vi "Test Client Alone With No Server.vi"(8 "error in (no error)":errorcluster) -> (0 "error out":errorcluster)   [LabVIEW 2019, in "RemoteControl.ZMQ.Tests.lvclass"]
uses:
  RemoteControl.ZMQ.Tests.lvclass
  C:/Program Files/National Instruments/LabVIEW 2019/user.lib/LevyLab/RemoteControl/RemoteControl/RemoteControl.lvclass
  <userlib>/LevyLab/RemoteControl/RemoteControl/RemoteControl.lvclass/RemoteControl.ctl
  <vilib>/numeric/Random Number (Range) U64.vi
  <vilib>/numeric/sub_Random U32.vi
  <vilib>/addons/_JKI Toolkits/Caraya/classes/Assert/Assert True.vi
  <userlib>/LevyLab/RemoteControl/RemoteControl/RemoteControl.lvclass
  <vilib>/addons/_JKI Toolkits/Caraya/classes/Assert/Assert.lvclass
  <vilib>/addons/_JKI Toolkits/Caraya/classes/Test/Test.lvclass
panel:
  out "code":i32
  out "Codes":i32[](array[numeric])
  in  "stop":bool
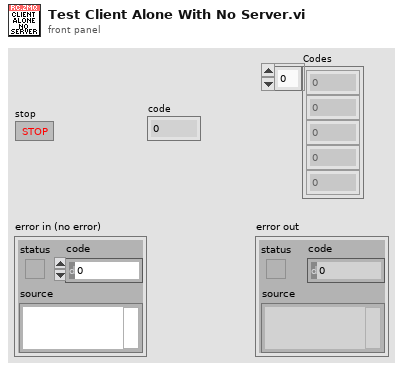
[diagram p1: front panel]
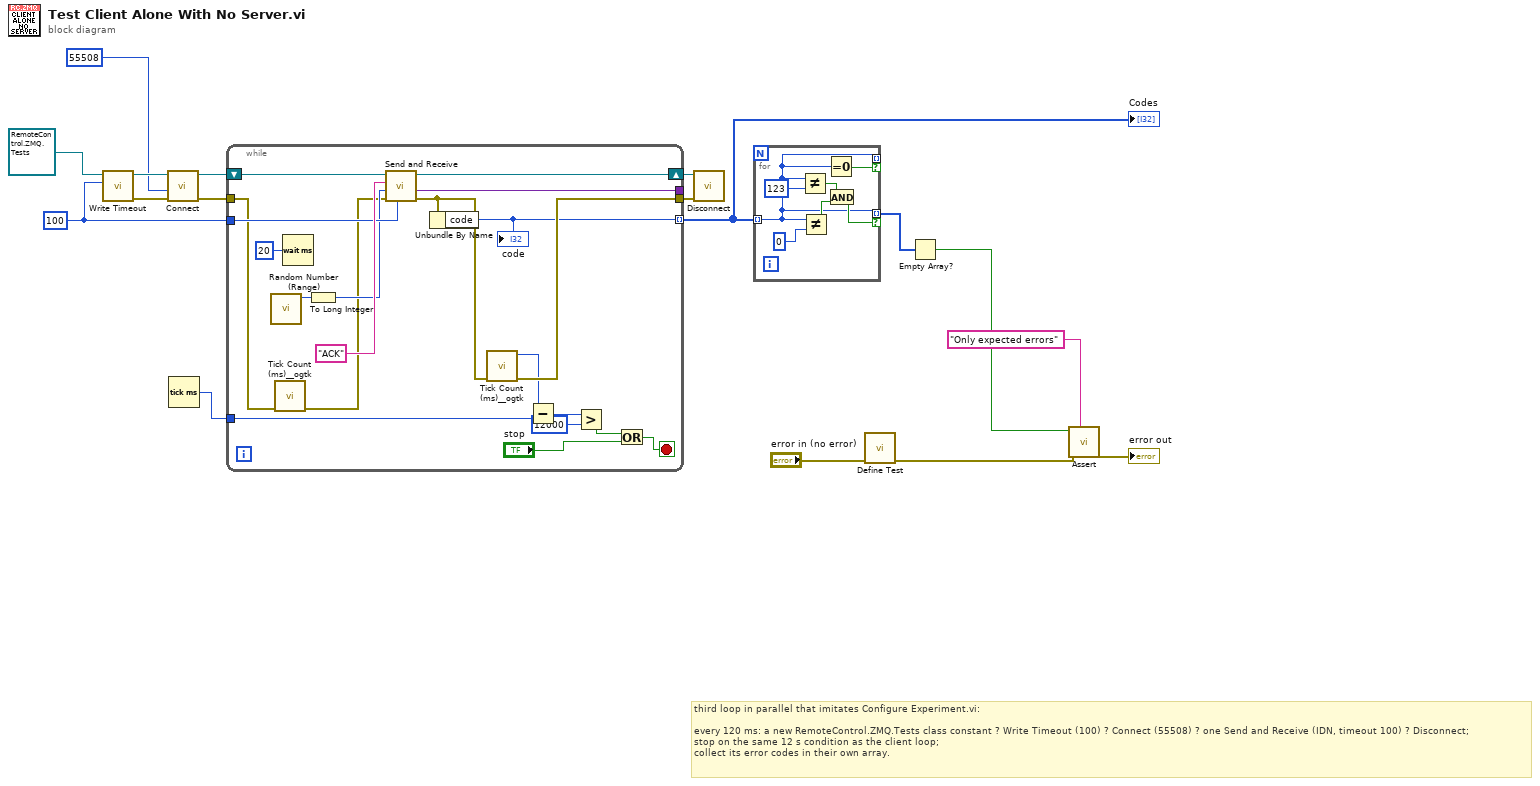
[diagram p0: block diagram]
diagram:
  w10 = 100 ("timeout in ms (100)")
  # "third loop in parallel that imitates Configure Experiment.vi:\n\nevery 120 ms: a new RemoteControl.ZMQ.Tests class constant ? Write Timeout (100) ? Connect (55508) ? one Send and Receive (IDN, timeout 100) ? Disconnect;\nstop on the same 12 s condition as the client loop;\ncollect its error codes in their own array."
  n1 = call <userlib>:"Write Timeout.vi"("timeout (ms) [500]"=w10, "RemoteControl in"=refnum<class "RemoteControl.ZMQ.Tests.lvclass"> refnum ("RemoteControl.ZMQ.Tests.lvclass")) -> ("error out"=w13:errorcluster, "RemoteControl out"=w12:refnum<class "RemoteControl.ZMQ.Tests.lvclass">)  [unwired: 8 in]
  n2 = call <userlib>:"Connect.vi"("error in (no error)"=w13, "Port"=u16 55508, "RemoteControl in"=w12) -> ("error out"=w15:errorcluster, "RemoteControl out"=w17:refnum<class "RemoteControl.ZMQ.Tests.lvclass">)  [unwired: 7 in]
  n3 = Tick Count (ms)() -> (millisecond timer value=w3:u32)
  n4 = while {
    tunnel: [w32] -> _
    tunnel: w10 -> [w33]
    shift-right: [w36] -> w16
    shift-left: w17 -> [w37]
    tunnel: w15 -> [w28]
    tunnel: [w26] -> w14
    tunnel: [w18] -> w5 mode=indexing
    tunnel: w3 -> [w24]
    stop <- w19 stop-if-true
    n5 = call-poly <vilib>:"Random Number (Range).vi"() -> ("number"=w35:u64)  [unwired: 11 in]
    n6 = call <userlib>:"Tick Count (ms)__ogtk.vi"("error in (no error)"=w28) -> ("error out"=w29:errorcluster)  [unwired: 9 in, 1 out]
    n7 = Wait (ms)(milliseconds to wait=u32 20) -> ()  [unwired: 1 out]
    n8 = To Long Integer(number=w35) -> (32bit integer=w31:i32)
    n9 = call <userlib>:"Send and Receive.vi"("timeout (ms) [500]"=w33, "error in (no error)"=w29, "Data"=w31, "Command"="ACK", "RemoteControl in"=w37) -> ("error out"=w27:errorcluster, "Data out"=w32:variant, "RemoteControl out"=w36:refnum<class "RemoteControl.ZMQ.Tests.lvclass">)  [unwired: 3 in, 1 out]
    n10 = Unbundle By Name(w27) -> ("code"=w18:i32)
    "code" <- w18
    n11 = call <userlib>:"Tick Count (ms)__ogtk.vi"("error in (no error)"=w27) -> ("error out"=w26:errorcluster, "millisecond timer value"=w25:u32)  [unwired: 9 in]
    n12 = Subtract(x=w25, y=w24) -> (x-y=w23:u32)
    n13 = Greater?(x=w23, y=u32 12000) -> (0:w21:bool)
    n14 = Or(x=w21, y="stop") -> (x .or. y?=w19:bool)
  }
  "Codes" <- w5
  n15 = call <userlib>:"Disconnect.vi"("error in (no error)"=w14, "RemoteControl in"=w16) -> ()  [unwired: 8 in, 2 out]
  n16 = for {
    tunnel: w5 -> [w39] mode=indexing
    tunnel: [w39] -> w8 mode=indexing if=w40
    tunnel: [w39] -> _ mode=indexing if=w38
    n17 = Not Equal?(x=w39, y=123) -> (x != y?=w42:bool)
    n18 = Not Equal?(x=w39, y=0) -> (x != y?=w41:bool)
    n19 = Equal To 0?(x=w39) -> (x = 0?=w38:bool)
    n20 = And(x=w42, y=w41) -> (x .and. y?=w40:bool)
  }
  n21 = call <vilib>:"Define Test.vi"("error in (no error)"="error in (no error)") -> ("error out"=w2:errorcluster)  [unwired: 9 in, 1 out]
  n22 = Empty Array?(array=w8) -> (empty?=w6:bool)
  n23 = call-poly <vilib>:"Assert.vi"("Label"="Only expected errors", "error in (no error)"=w2, "True?"=w6) -> ("error out"=→"error out":errorcluster)  [unwired: 7 in, 1 out]
